vi "Complete Multipart Upload.vi"(8 "error in (no error)":errorcluster, 11 "Multipart Upload":refnum<class "Multipart Upload.lvclass">) -> (0 "error out":errorcluster, 1 "ETag":string, 2 "Location":string, 3 "Bucket":refnum<class "Bucket.lvclass">, 4 "Version ID":string)   [LabVIEW 2015, in "NI_AWS_S3.lvlib" / "Multipart Upload.lvclass"]
uses:
  Multipart Upload.lvclass
  Bucket/Bucket.lvclass
  Core/HTTP Request/Name Value Pair.ctl
  Core/HTTP Request/Request Options.ctl
  Core/HTTP Request/Region handling.ctl
  Core/HTTP Request/URL formatting.ctl
  Multipart Upload.lvclass/Multipart Upload.ctl
  Bucket/Bucket.lvclass/Bucket.ctl
  Read Bucket.vi
  Read Upload ID.vi
  Read Object Key.vi
  Read Parts.vi
  Bucket/Read Name.vi
  Core/HTTP Request/HTTP Request.lvclass
  XML Parsing/NI_XML Parsing.lvlib
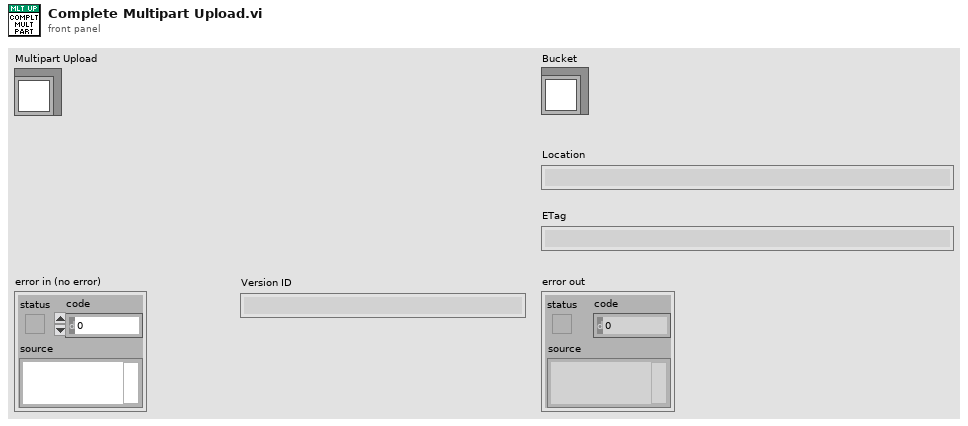
[diagram p1: front panel]
types:
  T1 = typedef "NI_AWS_Core.lvlib/HTTP Request.lvclass/Name Value Pair.ctl" = cluster{"name":string, "value":string}
  T2 = typedef "NI_AWS_Core.lvlib/HTTP Request.lvclass/Region handling.ctl" = enum16{"use region everywhere", "use region (authentication only)", "use region (URL only)", "ignore region everwhere"}
  T3 = typedef "NI_AWS_Core.lvlib/HTTP Request.lvclass/Request Options.ctl" = cluster{"request headers":T1[], "request parameters":T1[], "request body":string, "region handling":T2, "URL formatting":T4}
  T4 = typedef "NI_AWS_Core.lvlib/HTTP Request.lvclass/URL formatting.ctl" = enum16{"region-", "region."}
  T5 = typedef "NI_AWS_S3.lvlib/Part.ctl" = cluster{"Part Number":i32, "Last Modified":timestamp, "ETag":string, "Size":i32}
  T6 = typedef "NI_AWS_Core.lvlib/HTTP Request.lvclass/Response.ctl" = cluster{"Headers":string, "Body":string}
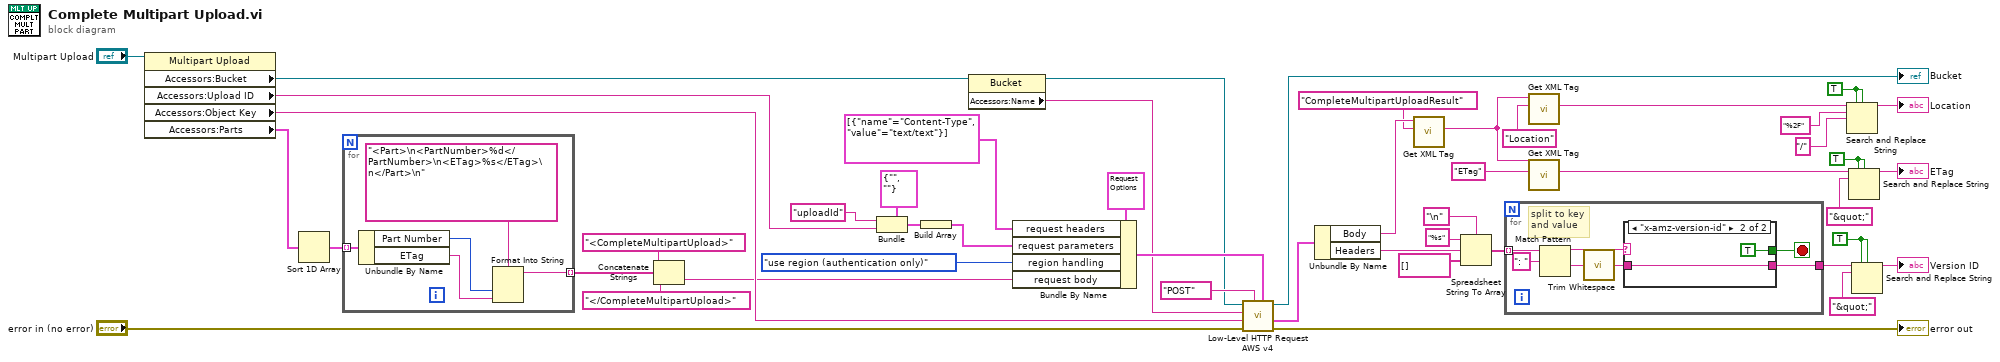
[diagram p0: block diagram]
diagram:
  w6 = TRUE ("replace all? (F)")
  w8 = TRUE ("replace all? (F)")
  w13 = TRUE ("replace all? (F)")
  n1 = property class="Multipart Upload"(reference="Multipart Upload") -> ("Accessors:Bucket"=w39:refnum<class "Bucket.lvclass">, "Accessors:Upload ID"=w33:string, "Accessors:Object Key"=w36:string, "Accessors:Parts"=w1:T5[])  [unwired: 1 in, 2 out]
  n2 = Sort 1D Array(array=w1) -> (sorted array=w30:T5[])
  n3 = for {
    tunnel: w30 -> [w53] mode=indexing
    tunnel: [w49] -> w31 mode=indexing
    n4 = Unbundle By Name(w53) -> ("Part Number"=w51:i32, "ETag"=w50:string)
    n5 = Format Into String(format string="<Part>\n<PartNumber>%d</PartNumber>\n<ETag>%s</ETag>\n</Part>\n", w51, w50) -> (resulting string=w49:string)  [unwired: 2 in, 1 out]
  }
  n6 = Concatenate Strings("<CompleteMultipartUpload>", w31, "</CompleteMultipartUpload>") -> (w27:string)
  n7 = Bundle(cluster=T1 {"name"="", "value"=""} ("Name Value Pair"), "name"="uploadId" ("format string"), "value"=w33) -> (w47:T1)
  n8 = Build Array(w47) -> (w34:T1[])
  n9 = property class="Bucket"(reference=w39) -> (reference out=w38:refnum<class "Bucket.lvclass">, "Accessors:Name"=w37:string)  [unwired: 1 in, 1 out]
  n10 = Bundle By Name(cluster=T3 {"request headers"=[], "request parameters"=[], "request body"="", "region handling"=enum."use region everywhere", "URL formatting"=enum."region."} ("Request Options"), "request headers"=T1[] [{"name"="Content-Type", "value"="text/text"}], "request parameters"=w34, "region handling"=Region_handling."use region (authentication only)", "request body"=w27) -> (w43:T3)
  n11 = call "Low-Level HTTP Request AWS v4.vi"("Request Options"=w43, "HTTP-Verb"="POST", "error in (no error)"="error in (no error)", "URL Suffix"=w36, "URL Prefix"=w37, "AWS Core in"=w38) -> ("error out"=→"error out":errorcluster, "Response"=w32:T6, "AWS Core out"=→"Bucket":refnum<class "Bucket.lvclass">)  [unwired: 2 in, 1 out]
  n12 = Unbundle By Name(w32) -> ("Body"=w20:string, "Headers"=w21:string)
  n13 = call "Get XML Tag.vi"("Tag name"="CompleteMultipartUploadResult", "XML String in"=w20) -> ("Tag value"=w17:string)  [unwired: 5 in, 4 out]
  n14 = Spreadsheet String To Array(delimiter (Tab)="\n", format string="%s", spreadsheet string=w21, array type (2D Dbl)=string[] []) -> (array=w23:string[])
  n15 = for {
    tunnel: w23 -> [w60] mode=indexing
    tunnel: [w54] -> w15
    stop <- w55 stop-if-true
    # "split to key\nand value"
    n16 = Match Pattern(string=w60, regular expression=": ") -> (before substring=w58:string, after substring=w57:string)  [unwired: 1 in, 2 out]
    n17 = call <vilib>:"Trim Whitespace.vi"("string"=w57) -> ("trimmed string"=w56:string)  [unwired: 1 in]
    n18 = case shown="\"x-amz-version-id\"" w58 {
      tunnel: w56 -> [_ w62]
      tunnel: [_ w62] -> w54
      tunnel: [_ TRUE] -> w55
      frame Default {
      }
      frame "x-amz-version-id" {
      }
    }
  }
  n19 = call "Get XML Tag.vi"("Tag name"="Location", "XML String in"=w17) -> ("Tag value"=w4:string)  [unwired: 5 in, 4 out]
  n20 = call "Get XML Tag.vi"("Tag name"="ETag", "XML String in"=w17) -> ("Tag value"=w10:string)  [unwired: 5 in, 4 out]
  n21 = Search and Replace String(replace all?=w6, case sensitive?=w6, input string=w4, search string="%2F", replace string="/") -> (result string=→"Location":string)  [unwired: 3 in, 3 out]
  n22 = Search and Replace String(replace all?=w8, case sensitive?=w8, input string=w10, search string="&quot;") -> (result string=→"ETag":string)  [unwired: 4 in, 3 out]
  n23 = Search and Replace String(replace all?=w13, case sensitive?=w13, input string=w15, search string="&quot;") -> (result string=→"Version ID":string)  [unwired: 4 in, 3 out]
